vi "Theta Calculation(SubVI).vi"(0 "User Input theta":dbl min=-45.0 max=45.0, 5 "Position=-85, I":dbl, 7 "Right":bool, 9 "Left":bool, 11 "User Input theta":refnum<vi>) -> (4 "Position=-85, O":dbl, 6 "Real output theta":dbl, 8 "Step diff":dbl)   [LabVIEW 2018]
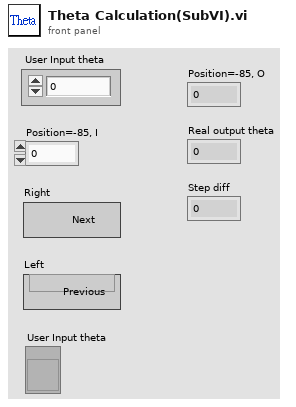
[diagram p1: front panel]
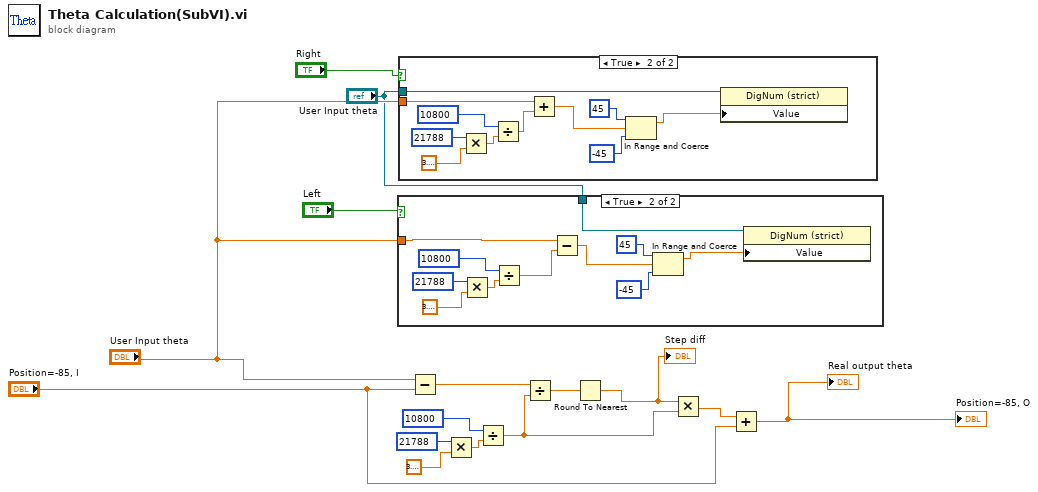
[diagram p0: block diagram]
diagram:
  n1 = case shown="True" "Left" {
    tunnel: "User Input theta" -> [_ w26]
    tunnel: "User Input theta" -> [_ w20]
    frame False {
    }
    frame True {
      n2 = Multiply(x=21788, y=3.141592653589793) -> (x*y=w24:dbl)
      n3 = Divide(x=10800, y=w24) -> (x/y=w21:dbl)
      n4 = Subtract(x=w26, y=w21) -> (x-y=w17:dbl)
      n5 = In Range and Coerce(upper limit=45, x=w17, lower limit=-45) -> (coerced(x)=w16:dbl)  [unwired: 1 out]
      n6 = property class="DigNum (strict)"(reference=w20, "Value"=w16) -> ()  [unwired: 1 in, 2 out]
    }
  }
  n7 = case shown="True" "Right" {
    tunnel: "User Input theta" -> [_ w35]
    tunnel: "User Input theta" -> [_ w31]
    frame False {
    }
    frame True {
      n8 = Multiply(x=21788, y=3.141592653589793) -> (x*y=w34:dbl)
      n9 = Divide(x=10800, y=w34) -> (x/y=w36:dbl)
      n10 = Add(x=w35, y=w36) -> (x+y=w28:dbl)
      n11 = In Range and Coerce(upper limit=45, x=w28, lower limit=-45) -> (coerced(x)=w27:dbl)  [unwired: 1 out]
      n12 = property class="DigNum (strict)"(reference=w31, "Value"=w27) -> ()  [unwired: 1 in, 2 out]
    }
  }
  n13 = Subtract(x="User Input theta", y="Position=-85, I") -> (x-y=w7:dbl)
  n14 = Multiply(x=21788, y=3.141592653589793) -> (x*y=w4:dbl)
  n15 = Divide(x=10800, y=w4) -> (x/y=w9:dbl)
  n16 = Divide(x=w7, y=w9) -> (x/y=w8:dbl)
  n17 = Round To Nearest(number=w8) -> (nearest integer value=w11:dbl)
  "Step diff" <- w11
  n18 = Multiply(x=w11, y=w9) -> (x*y=w2:dbl)
  n19 = Add(x=w2, y="Position=-85, I") -> (x+y=→"Real output theta" →"Position=-85, O":dbl)
